vi "Read Month.vi"(7 "Time Entry Store in":refnum<class "Time Entry Store-INI.lvclass">, 8 "error in (no error)":errorcluster, 10 "Month":i32, 11 "Year":i32) -> (0 "error out":errorcluster, 3 "Time Entries":T1, 5 "Time Entry Store out":refnum<class "Time Entry Store-INI.lvclass">)   [LabVIEW 2024, in "Time Entry Store-INI.lvclass"]
doc: "Returns every time entry in the month file YYYY-MM.ini for the given year and month - the entries whose Start Time falls in that month in UTC - sorted by Start Time. A month without a file returns an empty array.\n\nGenerated by: Claude"
uses:
  Time Entry Store-INI.lvclass
  Time Entry Store-INI.lvclass/Time Entry Store-INI.ctl
  Rows/Time Entry.ctl
  Rows/Time Entry List.ctl
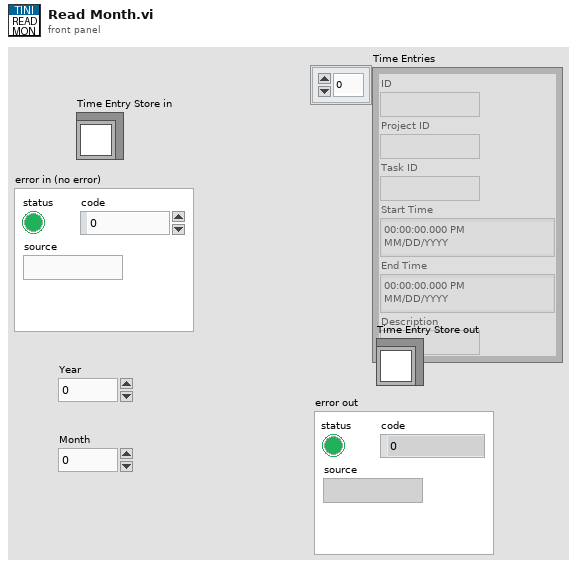
[diagram p1: front panel]
types:
  T1 = typedef "Time Entry List.ctl" = T2[]
  T2 = typedef "Time Entry.ctl" = cluster{"ID":string, "Project ID":string, "Task ID":string, "Start Time":timestamp, "End Time":timestamp, "Description":string}
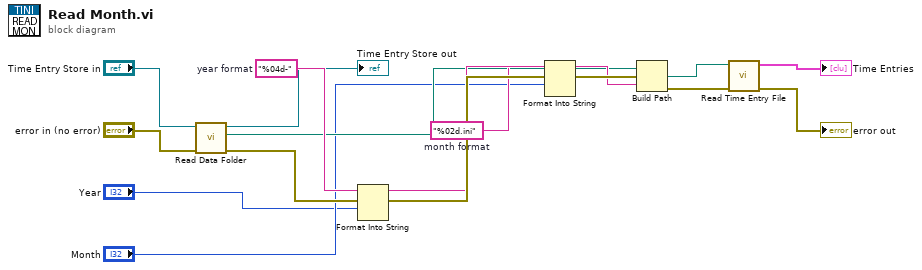
[diagram p0: block diagram]
diagram:
  w9 = "%02d.ini"  # month format
  w8 = "%04d-"  # year format
  n1 = call-dynamic "Read Data Folder.vi"("error in (no error)"="error in (no error)", "Time Entry Store-INI in"="Time Entry Store in") -> ("error out"=w5:errorcluster, "Data Folder"=w7:path, "Time Entry Store-INI out"=→"Time Entry Store out":refnum<class "Time Entry Store-INI.lvclass">)  [unwired: 7 in]
  n2 = Format Into String(format string=w8, error in=w5, "Year") -> (resulting string=w10:string, error out=w11:errorcluster)  [unwired: 1 in]
  n3 = Format Into String(format string=w9, initial string=w10, error in=w11, "Month") -> (resulting string=w12:string, error out=w13:errorcluster)
  n4 = Build Path(base path=w7, name or relative path=w12) -> (appended path=w14:path)
  n5 = call "Read Time Entry File.vi"("error in (no error)"=w13, "File Path"=w14) -> ("error out"=→"error out":errorcluster, "Time Entries"=→"Time Entries":T1)  [unwired: 6 in, 2 out]
